vi "input.vi"(8 "error in":errorcluster, 10 "data table in":T1, 11 "Scan Engine runtime in":refnum<class "Scan Engine runtime.lvclass">) -> (0 "error out":errorcluster, 2 "data table out":T1, 3 "Scan Engine runtime out":refnum<class "Scan Engine runtime.lvclass">)   [LabVIEW 2015, in "Scan Engine runtime.lvclass"]
doc: "Provides an interface for reading data from a module at runtime. While this interface performs no operations, a child should provide an override which may read from any open sessions, references, or interfaces."
uses:
  Scan Engine runtime.lvclass
  <vilib>/NI/Tag Bus/table/data table.ctl
  Scan Engine runtime.lvclass/Scan Engine runtime.ctl
  <vilib>/NI/Tag Bus/table/data polymorphs/write one/write Double.vi
  <vilib>/NI/Tag Bus/table/data polymorphs/write one/write Single.vi
  <vilib>/NI/Tag Bus/table/data polymorphs/write one/write I64.vi
  <vilib>/NI/Tag Bus/table/data polymorphs/write one/write I32.vi
  <vilib>/NI/Tag Bus/table/data polymorphs/write one/write I16.vi
  <vilib>/NI/Tag Bus/table/data polymorphs/write one/write I8.vi
  <vilib>/NI/Tag Bus/table/data polymorphs/write one/write U64.vi
  <vilib>/NI/Tag Bus/table/data polymorphs/write one/write U32.vi
  <vilib>/NI/Tag Bus/table/data polymorphs/write one/write U16.vi
  <vilib>/NI/Tag Bus/table/data polymorphs/write one/write U8.vi
  <vilib>/NI/Tag Bus/table/data polymorphs/write one/write Boolean.vi
  <vilib>/NI/Tag Bus/table/data polymorphs/write many/write Doubles.vi
  <vilib>/NI/Tag Bus/table/data polymorphs/write many/write Singles.vi
  <vilib>/NI/Tag Bus/table/data polymorphs/write many/write I64s.vi
  <vilib>/NI/Tag Bus/table/data polymorphs/write many/write I32s.vi
  <vilib>/NI/Tag Bus/table/data polymorphs/write many/write I16s.vi
  <vilib>/NI/Tag Bus/table/data polymorphs/write many/write I8s.vi
  <vilib>/NI/Tag Bus/table/data polymorphs/write many/write U64s.vi
  <vilib>/NI/Tag Bus/table/data polymorphs/write many/write U32s.vi
  <vilib>/NI/Tag Bus/table/data polymorphs/write many/write U16s.vi
  <vilib>/NI/Tag Bus/table/data polymorphs/write many/write U8s.vi
  <vilib>/NI/Tag Bus/table/data polymorphs/write many/write Booleans.vi
  <vilib>/NI/Tag Bus/table/data table.lvlib
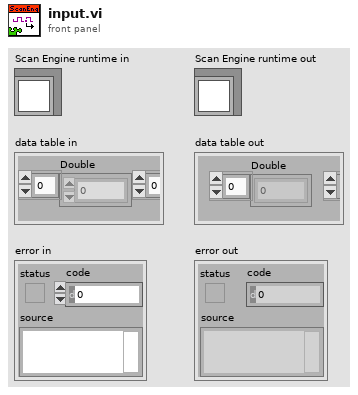
[diagram p1: front panel]
types:
  T1 = typedef "tag bus.lvlib/data table.lvlib/data table.ctl" = cluster{"Double":dbl[], "Single":sgl[], "I64":i64[], "I32":i32[], "I16":i16[], "I8":i8[], "U64":u64[], "U32":u32[], "U16":u16[], "U8":u8[], "Boolean":bool[], "String":string[], "Array of Double":cluster{"DBL Array":dbl[]}[], "Array of Single":cluster{"SGL Array":sgl[]}[], "Array of I64":cluster{"I64 Array":i64[]}[], "Array of I32":cluster{"I32 Array":i32[]}[], "Array of I16":cluster{"I16 Array":i16[]}[], "Array of I8":cluster{"I8 Array":i8[]}[], "Array of U64":cluster{"U64 Array":u64[]}[], "Array of U32":cluster{"U32 Array":u32[]}[], "Array of U16":cluster{"U16 Array":u16[]}[], "Array of U8":cluster{"U8 Array":u8[]}[], "Array of Boolean":cluster{"Boolean Array":bool[]}[], "Array of String":cluster{"String Array":string[]}[]}
  T2 = typedef "Scan Engine runtime.lvclass/IO_index_map.ctl" = cluster{"module_ref":refnum<k21>, "data type":T3, "IO_variable_info":T4[], "IO_module_index_array":i32[], "IO_table_index":i32[], "IO_table_index_ordered":i32[], "use_scanned_methods":bool}
  T3 = typedef "tag bus.lvlib/tag descriptor.lvclass/Data Type.ctl" = enum16{"Double", "Single", "I64", "I32", "I16", "I8", "U64", "U32", "U16", "U8", "Boolean", "String", "Array of Double", "Array of Single", "Array of I64", "Array of I32", "Array of I16", "Array of I8", "Array of U64", "Array of U32", "Array of U16", "Array of U8", "Array of Boolean", "Array of String"}
  T4 = typedef "Scan Engine runtime.lvclass/Index Map.ctl" = cluster{"data type":T3, "variable ref":refnum<k21>, "index":i32, "IO Var":bool, "module_index":i32}
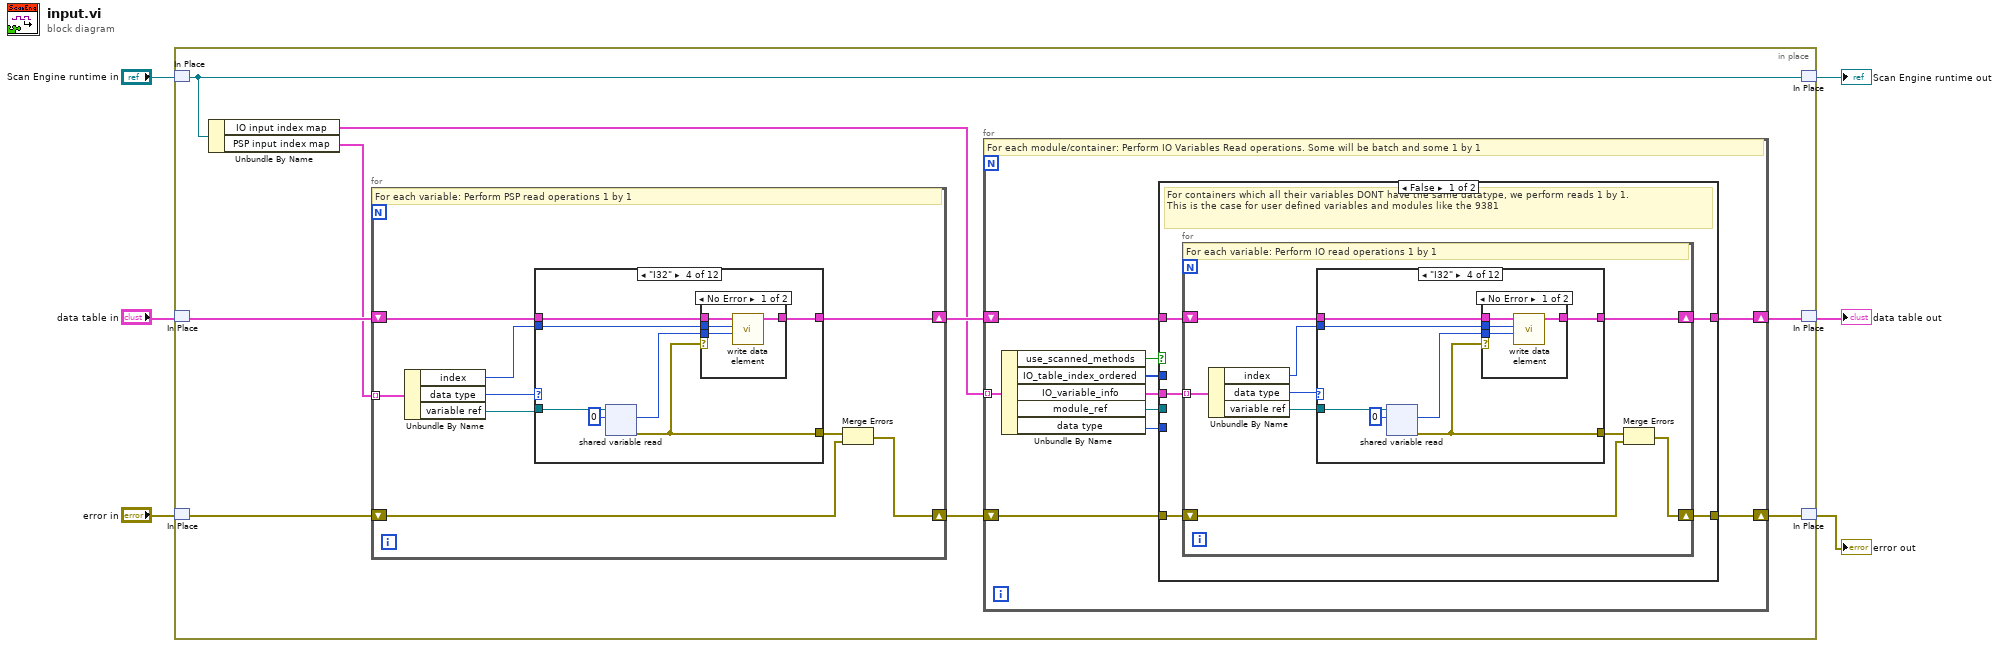
[diagram p0: block diagram]
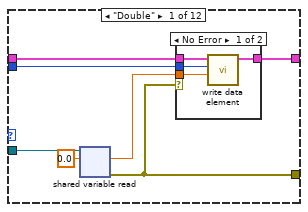
[diagram p2: hidden frame]
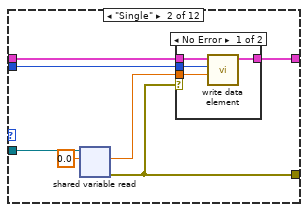
[diagram p4: hidden frame]
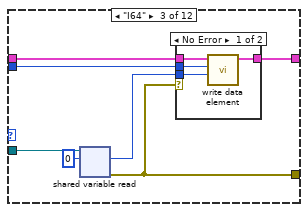
[diagram p6: hidden frame]
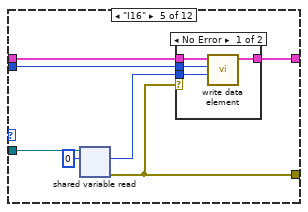
[diagram p9: hidden frame]
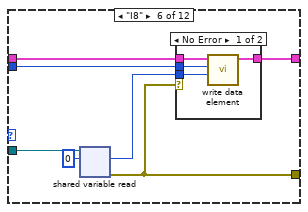
[diagram p11: hidden frame]
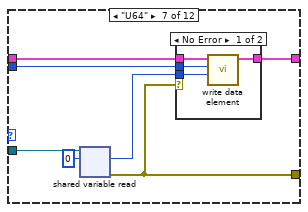
[diagram p13: hidden frame]
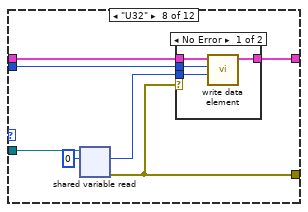
[diagram p15: hidden frame]
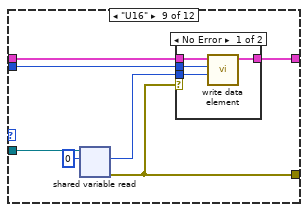
[diagram p17: hidden frame]
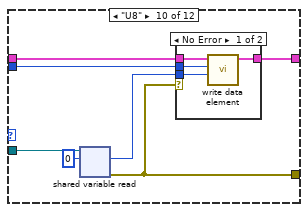
[diagram p19: hidden frame]
diagram:
  n1 = in-place {
    n2 = in-place-match #1("Scan Engine runtime in") -> (w15:refnum<class "Scan Engine runtime.lvclass">)
    n3 = in-place-match #2("data table in") -> (w14:T1)
    n4 = in-place-match #3("error in") -> (w13:errorcluster)
    n5 = Unbundle By Name(w15) -> ("IO input index map"=w10:T2[], "PSP input index map"=w9:T4[])
    n6 = for {
      shift-right: [w267] -> w12
      shift-left: w14 -> [w268]
      shift-right: [w262] -> w8
      shift-left: w13 -> [w263]
      tunnel: w9 -> [w270] mode=indexing
      # "For each variable: Perform PSP read operations 1 by 1"
      n7 = Unbundle By Name(w270) -> ("index"=w266:i32, "data type"=w269:T3, "variable ref"=w265:refnum<k21>)
      n8 = case shown="\"I32\"" w269 {
        tunnel: w268 -> [w277 w289 w301 w313 w325 w337 w349 w361 w373 w385 w397 w404]
        tunnel: [w276 w288 w300 w312 w324 w336 w348 w360 w372 w384 w396 w404] -> w267
        tunnel: w266 -> [w275 w287 w299 w311 w323 w335 w347 w359 w371 w383 w395 _]
        tunnel: w265 -> [w274 w286 w298 w310 w322 w334 w346 w358 w370 w382 w394 _]
        tunnel: [w271 w283 w295 w307 w319 w331 w343 w355 w367 w379 w391 errorcluster {"status"=FALSE, "code"=0, "source"=""} ("error IO")] -> w264
        frame "Double" {
          n9 = shared-variable-read(w274, 0.0) -> (w271:errorcluster, w272:dbl)  [unwired: 1 in, 1 out]
          n10 = case shown="No Error" w271 {
            tunnel: w277 -> [w281 w282]
            tunnel: [w280 w282] -> w276
            tunnel: w275 -> [w279 _]
            tunnel: w272 -> [w278 _]
            frame No Error {
              n11 = call-poly <vilib>:"write data element.vi"("value"=w278, "index"=w279, "data table in"=w281) -> ("data table out"=w280:T1)  [unwired: 8 in]
            }
            frame Error {
            }
          }
        }
        frame "Single" {
          n12 = shared-variable-read(w286, sgl 0.0) -> (w283:errorcluster, w284:sgl)  [unwired: 1 in, 1 out]
          n13 = case shown="No Error" w283 {
            tunnel: w289 -> [w293 w294]
            tunnel: [w292 w294] -> w288
            tunnel: w287 -> [w291 _]
            tunnel: w284 -> [w290 _]
            frame No Error {
              n14 = call-poly <vilib>:"write data element.vi"("value"=w290, "index"=w291, "data table in"=w293) -> ("data table out"=w292:T1)  [unwired: 8 in]
            }
            frame Error {
            }
          }
        }
        frame "I64" {
          n15 = shared-variable-read(w298, i64 0) -> (w295:errorcluster, w296:i64)  [unwired: 1 in, 1 out]
          n16 = case shown="No Error" w295 {
            tunnel: w301 -> [w305 w306]
            tunnel: [w304 w306] -> w300
            tunnel: w299 -> [w303 _]
            tunnel: w296 -> [w302 _]
            frame No Error {
              n17 = call-poly <vilib>:"write data element.vi"("value"=w302, "index"=w303, "data table in"=w305) -> ("data table out"=w304:T1)  [unwired: 8 in]
            }
            frame Error {
            }
          }
        }
        frame "I32" {
          n18 = shared-variable-read(w310, 0) -> (w307:errorcluster, w308:i32)  [unwired: 1 in, 1 out]
          n19 = case shown="No Error" w307 {
            tunnel: w313 -> [w317 w318]
            tunnel: [w316 w318] -> w312
            tunnel: w311 -> [w315 _]
            tunnel: w308 -> [w314 _]
            frame No Error {
              n20 = call-poly <vilib>:"write data element.vi"("value"=w314, "index"=w315, "data table in"=w317) -> ("data table out"=w316:T1)  [unwired: 8 in]
            }
            frame Error {
            }
          }
        }
        frame "I16" {
          n21 = shared-variable-read(w322, i16 0) -> (w319:errorcluster, w320:i16)  [unwired: 1 in, 1 out]
          n22 = case shown="No Error" w319 {
            tunnel: w325 -> [w329 w330]
            tunnel: [w328 w330] -> w324
            tunnel: w323 -> [w327 _]
            tunnel: w320 -> [w326 _]
            frame No Error {
              n23 = call-poly <vilib>:"write data element.vi"("value"=w326, "index"=w327, "data table in"=w329) -> ("data table out"=w328:T1)  [unwired: 8 in]
            }
            frame Error {
            }
          }
        }
        frame "I8" {
          n24 = shared-variable-read(w334, i8 0) -> (w331:errorcluster, w332:i8)  [unwired: 1 in, 1 out]
          n25 = case shown="No Error" w331 {
            tunnel: w337 -> [w341 w342]
            tunnel: [w340 w342] -> w336
            tunnel: w335 -> [w339 _]
            tunnel: w332 -> [w338 _]
            frame No Error {
              n26 = call-poly <vilib>:"write data element.vi"("value"=w338, "index"=w339, "data table in"=w341) -> ("data table out"=w340:T1)  [unwired: 8 in]
            }
            frame Error {
            }
          }
        }
        frame "U64" {
          n27 = shared-variable-read(w346, u64 0) -> (w343:errorcluster, w344:u64)  [unwired: 1 in, 1 out]
          n28 = case shown="No Error" w343 {
            tunnel: w349 -> [w353 w354]
            tunnel: [w352 w354] -> w348
            tunnel: w347 -> [w351 _]
            tunnel: w344 -> [w350 _]
            frame No Error {
              n29 = call-poly <vilib>:"write data element.vi"("value"=w350, "index"=w351, "data table in"=w353) -> ("data table out"=w352:T1)  [unwired: 8 in]
            }
            frame Error {
            }
          }
        }
        frame "U32" {
          n30 = shared-variable-read(w358, u32 0) -> (w355:errorcluster, w356:u32)  [unwired: 1 in, 1 out]
          n31 = case shown="No Error" w355 {
            tunnel: w361 -> [w365 w366]
            tunnel: [w364 w366] -> w360
            tunnel: w359 -> [w363 _]
            tunnel: w356 -> [w362 _]
            frame No Error {
              n32 = call-poly <vilib>:"write data element.vi"("value"=w362, "index"=w363, "data table in"=w365) -> ("data table out"=w364:T1)  [unwired: 8 in]
            }
            frame Error {
            }
          }
        }
        frame "U16" {
          n33 = shared-variable-read(w370, u16 0) -> (w367:errorcluster, w368:u16)  [unwired: 1 in, 1 out]
          n34 = case shown="No Error" w367 {
            tunnel: w373 -> [w377 w378]
            tunnel: [w376 w378] -> w372
            tunnel: w371 -> [w375 _]
            tunnel: w368 -> [w374 _]
            frame No Error {
              n35 = call-poly <vilib>:"write data element.vi"("value"=w374, "index"=w375, "data table in"=w377) -> ("data table out"=w376:T1)  [unwired: 8 in]
            }
            frame Error {
            }
          }
        }
        frame "U8" {
          n36 = shared-variable-read(w382, u8 0) -> (w379:errorcluster, w380:u8)  [unwired: 1 in, 1 out]
          n37 = case shown="No Error" w379 {
            tunnel: w385 -> [w389 w390]
            tunnel: [w388 w390] -> w384
            tunnel: w383 -> [w387 _]
            tunnel: w380 -> [w386 _]
            frame No Error {
              n38 = call-poly <vilib>:"write data element.vi"("value"=w386, "index"=w387, "data table in"=w389) -> ("data table out"=w388:T1)  [unwired: 8 in]
            }
            frame Error {
            }
          }
        }
        frame "Boolean" {
          n39 = shared-variable-read(w394, FALSE) -> (w391:errorcluster, w392:bool)  [unwired: 1 in, 1 out]
          n40 = case shown="No Error" w391 {
            tunnel: w397 -> [w401 w402]
            tunnel: [w400 w402] -> w396
            tunnel: w395 -> [w399 _]
            tunnel: w392 -> [w398 _]
            frame No Error {
              n41 = call-poly <vilib>:"write data element.vi"("value"=w398, "index"=w399, "data table in"=w401) -> ("data table out"=w400:T1)  [unwired: 8 in]
            }
            frame Error {
            }
          }
        }
        frame Default {
        }
      }
      n42 = Merge Errors(w264, w263) -> (w262:errorcluster)
    }
    n43 = for {
      shift-right: [w23] -> w11
      shift-left: w12 -> [w24]
      shift-right: [w21] -> w7
      shift-left: w8 -> [w22]
      tunnel: w10 -> [w25] mode=indexing
      # "For each module/container: Perform IO Variables Read operations. Some will be batch and some 1 by 1"
      n44 = Unbundle By Name(w25) -> ("use_scanned_methods"=w16:bool, "IO_table_index_ordered"=w18:i32[], "IO_variable_info"=w17:T4[], "module_ref"=w20:refnum<k21>, "data type"=w19:T3)
      n45 = case shown="False" w16 {
        tunnel: w24 -> [w26 w182]
        tunnel: [w27 w181] -> w23
        tunnel: w22 -> [w29 w179]
        tunnel: [w28 w178] -> w21
        tunnel: w20 -> [_ w177]
        tunnel: w19 -> [_ w176]
        tunnel: w18 -> [_ w175]
        tunnel: w17 -> [w30 w174]
        frame False {
          # "For containers which all their variables DONT have the same datatype, we perform reads 1 by 1.\nThis is the case for user defined variables and modules like the 9381"
          n46 = for {
            shift-right: [w36] -> w27
            shift-left: w26 -> [w37]
            shift-right: [w31] -> w28
            shift-left: w29 -> [w32]
            tunnel: w30 -> [w39] mode=indexing
            # "For each variable: Perform IO read operations 1 by 1"
            n47 = Unbundle By Name(w39) -> ("index"=w35:i32, "data type"=w38:T3, "variable ref"=w34:refnum<k21>)
            n48 = case shown="\"I32\"" w38 {
              tunnel: w37 -> [w46 w58 w70 w82 w94 w106 w118 w130 w142 w154 w166 w173]
              tunnel: [w45 w57 w69 w81 w93 w105 w117 w129 w141 w153 w165 w173] -> w36
              tunnel: w35 -> [w44 w56 w68 w80 w92 w104 w116 w128 w140 w152 w164 _]
              tunnel: w34 -> [w43 w55 w67 w79 w91 w103 w115 w127 w139 w151 w163 _]
              tunnel: [w40 w52 w64 w76 w88 w100 w112 w124 w136 w148 w160 errorcluster {"status"=FALSE, "code"=0, "source"=""} ("error IO")] -> w33
              frame "Double" {
                n49 = shared-variable-read(w43, 0.0) -> (w40:errorcluster, w41:dbl)  [unwired: 1 in, 1 out]
                n50 = case shown="No Error" w40 {
                  tunnel: w46 -> [w50 w51]
                  tunnel: [w49 w51] -> w45
                  tunnel: w44 -> [w48 _]
                  tunnel: w41 -> [w47 _]
                  frame No Error {
                    n51 = call-poly <vilib>:"write data element.vi"("value"=w47, "index"=w48, "data table in"=w50) -> ("data table out"=w49:T1)  [unwired: 8 in]
                  }
                  frame Error {
                  }
                }
              }
              frame "Single" {
                n52 = shared-variable-read(w55, sgl 0.0) -> (w52:errorcluster, w53:sgl)  [unwired: 1 in, 1 out]
                n53 = case shown="No Error" w52 {
                  tunnel: w58 -> [w62 w63]
                  tunnel: [w61 w63] -> w57
                  tunnel: w56 -> [w60 _]
                  tunnel: w53 -> [w59 _]
                  frame No Error {
                    n54 = call-poly <vilib>:"write data element.vi"("value"=w59, "index"=w60, "data table in"=w62) -> ("data table out"=w61:T1)  [unwired: 8 in]
                  }
                  frame Error {
                  }
                }
              }
              frame "I64" {
                n55 = shared-variable-read(w67, i64 0) -> (w64:errorcluster, w65:i64)  [unwired: 1 in, 1 out]
                n56 = case shown="No Error" w64 {
                  tunnel: w70 -> [w74 w75]
                  tunnel: [w73 w75] -> w69
                  tunnel: w68 -> [w72 _]
                  tunnel: w65 -> [w71 _]
                  frame No Error {
                    n57 = call-poly <vilib>:"write data element.vi"("value"=w71, "index"=w72, "data table in"=w74) -> ("data table out"=w73:T1)  [unwired: 8 in]
                  }
                  frame Error {
                  }
                }
              }
              frame "I32" {
                n58 = shared-variable-read(w79, 0) -> (w76:errorcluster, w77:i32)  [unwired: 1 in, 1 out]
                n59 = case shown="No Error" w76 {
                  tunnel: w82 -> [w86 w87]
                  tunnel: [w85 w87] -> w81
                  tunnel: w80 -> [w84 _]
                  tunnel: w77 -> [w83 _]
                  frame No Error {
                    n60 = call-poly <vilib>:"write data element.vi"("value"=w83, "index"=w84, "data table in"=w86) -> ("data table out"=w85:T1)  [unwired: 8 in]
                  }
                  frame Error {
                  }
                }
              }
              frame "I16" {
                n61 = shared-variable-read(w91, i16 0) -> (w88:errorcluster, w89:i16)  [unwired: 1 in, 1 out]
                n62 = case shown="No Error" w88 {
                  tunnel: w94 -> [w98 w99]
                  tunnel: [w97 w99] -> w93
                  tunnel: w92 -> [w96 _]
                  tunnel: w89 -> [w95 _]
                  frame No Error {
                    n63 = call-poly <vilib>:"write data element.vi"("value"=w95, "index"=w96, "data table in"=w98) -> ("data table out"=w97:T1)  [unwired: 8 in]
                  }
                  frame Error {
                  }
                }
              }
              frame "I8" {
                n64 = shared-variable-read(w103, i8 0) -> (w100:errorcluster, w101:i8)  [unwired: 1 in, 1 out]
                n65 = case shown="No Error" w100 {
                  tunnel: w106 -> [w110 w111]
                  tunnel: [w109 w111] -> w105
                  tunnel: w104 -> [w108 _]
                  tunnel: w101 -> [w107 _]
                  frame No Error {
                    n66 = call-poly <vilib>:"write data element.vi"("value"=w107, "index"=w108, "data table in"=w110) -> ("data table out"=w109:T1)  [unwired: 8 in]
                  }
                  frame Error {
                  }
                }
              }
              frame "U64" {
                n67 = shared-variable-read(w115, u64 0) -> (w112:errorcluster, w113:u64)  [unwired: 1 in, 1 out]
                n68 = case shown="No Error" w112 {
                  tunnel: w118 -> [w122 w123]
                  tunnel: [w121 w123] -> w117
                  tunnel: w116 -> [w120 _]
                  tunnel: w113 -> [w119 _]
                  frame No Error {
                    n69 = call-poly <vilib>:"write data element.vi"("value"=w119, "index"=w120, "data table in"=w122) -> ("data table out"=w121:T1)  [unwired: 8 in]
                  }
                  frame Error {
                  }
                }
              }
              frame "U32" {
                n70 = shared-variable-read(w127, u32 0) -> (w124:errorcluster, w125:u32)  [unwired: 1 in, 1 out]
                n71 = case shown="No Error" w124 {
                  tunnel: w130 -> [w134 w135]
                  tunnel: [w133 w135] -> w129
                  tunnel: w128 -> [w132 _]
                  tunnel: w125 -> [w131 _]
                  frame No Error {
                    n72 = call-poly <vilib>:"write data element.vi"("value"=w131, "index"=w132, "data table in"=w134) -> ("data table out"=w133:T1)  [unwired: 8 in]
                  }
                  frame Error {
                  }
                }
              }
              frame "U16" {
                n73 = shared-variable-read(w139, u16 0) -> (w136:errorcluster, w137:u16)  [unwired: 1 in, 1 out]
                n74 = case shown="No Error" w136 {
                  tunnel: w142 -> [w146 w147]
                  tunnel: [w145 w147] -> w141
                  tunnel: w140 -> [w144 _]
                  tunnel: w137 -> [w143 _]
                  frame No Error {
                    n75 = call-poly <vilib>:"write data element.vi"("value"=w143, "index"=w144, "data table in"=w146) -> ("data table out"=w145:T1)  [unwired: 8 in]
                  }
                  frame Error {
                  }
                }
              }
              frame "U8" {
                n76 = shared-variable-read(w151, u8 0) -> (w148:errorcluster, w149:u8)  [unwired: 1 in, 1 out]
                n77 = case shown="No Error" w148 {
                  tunnel: w154 -> [w158 w159]
                  tunnel: [w157 w159] -> w153
                  tunnel: w152 -> [w156 _]
                  tunnel: w149 -> [w155 _]
                  frame No Error {
                    n78 = call-poly <vilib>:"write data element.vi"("value"=w155, "index"=w156, "data table in"=w158) -> ("data table out"=w157:T1)  [unwired: 8 in]
                  }
                  frame Error {
                  }
                }
              }
              frame "Boolean" {
                n79 = shared-variable-read(w163, FALSE) -> (w160:errorcluster, w161:bool)  [unwired: 1 in, 1 out]
                n80 = case shown="No Error" w160 {
                  tunnel: w166 -> [w170 w171]
                  tunnel: [w169 w171] -> w165
                  tunnel: w164 -> [w168 _]
                  tunnel: w161 -> [w167 _]
                  frame No Error {
                    n81 = call-poly <vilib>:"write data element.vi"("value"=w167, "index"=w168, "data table in"=w170) -> ("data table out"=w169:T1)  [unwired: 8 in]
                  }
                  frame Error {
                  }
                }
              }
              frame Default {
              }
            }
            n82 = Merge Errors(w33, w32) -> (w31:errorcluster)
          }
        }
        frame True {
          # "For containers which all their variables have the same datatype, we perform a batch read"
          n83 = case shown="\"Single\"" w176 {
            tunnel: w182 -> [w185 w192 w199 w206 w213 w220 w227 w234 w241 w248 w255 w261]
            tunnel: [w186 w193 w200 w207 w214 w221 w228 w235 w242 w249 w256 w261] -> w181
            tunnel: w177 -> [w189 w196 w203 w210 w217 w224 w231 w238 w245 w252 w259 _]
            tunnel: [w188 w195 w202 w209 w216 w223 w230 w237 w244 w251 w258 errorcluster {"status"=FALSE, "code"=0, "source"=""} ("error IO")] -> w180
            tunnel: w175 -> [w184 w191 w198 w205 w212 w219 w226 w233 w240 w247 w254 _]
            tunnel: w174 -> [_ _ _ _ _ _ _ _ _ _ _ _]
            frame "Double" {
              n84 = shared-variable-read(w189, dbl[] []) -> (w188:errorcluster, w183:dbl[])  [unwired: 1 in, 1 out]
              n85 = call-poly <vilib>:"write multiple elements.vi"("values"=w183, "indices"=w184, "data table in"=w185) -> ("data table out"=w186:T1)  [unwired: 8 in]
            }
            frame "Single" {
              n86 = shared-variable-read(w196, sgl[] []) -> (w195:errorcluster, w190:sgl[])  [unwired: 1 in, 1 out]
              n87 = call-poly <vilib>:"write multiple elements.vi"("values"=w190, "indices"=w191, "data table in"=w192) -> ("data table out"=w193:T1)  [unwired: 8 in]
            }
            frame "I64" {
              n88 = shared-variable-read(w203, i64[] []) -> (w202:errorcluster, w197:i64[])  [unwired: 1 in, 1 out]
              n89 = call-poly <vilib>:"write multiple elements.vi"("values"=w197, "indices"=w198, "data table in"=w199) -> ("data table out"=w200:T1)  [unwired: 8 in]
            }
            frame "I32" {
              n90 = shared-variable-read(w210, i32[] []) -> (w209:errorcluster, w204:i32[])  [unwired: 1 in, 1 out]
              n91 = call-poly <vilib>:"write multiple elements.vi"("values"=w204, "indices"=w205, "data table in"=w206) -> ("data table out"=w207:T1)  [unwired: 8 in]
            }
            frame "I16" {
              n92 = shared-variable-read(w217, i16[] []) -> (w216:errorcluster, w211:i16[])  [unwired: 1 in, 1 out]
              n93 = call-poly <vilib>:"write multiple elements.vi"("values"=w211, "indices"=w212, "data table in"=w213) -> ("data table out"=w214:T1)  [unwired: 8 in]
            }
            frame "I8" {
              n94 = shared-variable-read(w224, i8[] []) -> (w223:errorcluster, w218:i8[])  [unwired: 1 in, 1 out]
              n95 = call-poly <vilib>:"write multiple elements.vi"("values"=w218, "indices"=w219, "data table in"=w220) -> ("data table out"=w221:T1)  [unwired: 8 in]
            }
            frame "U64" {
              n96 = shared-variable-read(w231, u64[] []) -> (w230:errorcluster, w225:u64[])  [unwired: 1 in, 1 out]
              n97 = call-poly <vilib>:"write multiple elements.vi"("values"=w225, "indices"=w226, "data table in"=w227) -> ("data table out"=w228:T1)  [unwired: 8 in]
            }
            frame "U32" {
              n98 = shared-variable-read(w238, u32[] []) -> (w237:errorcluster, w232:u32[])  [unwired: 1 in, 1 out]
              n99 = call-poly <vilib>:"write multiple elements.vi"("values"=w232, "indices"=w233, "data table in"=w234) -> ("data table out"=w235:T1)  [unwired: 8 in]
            }
            frame "U16" {
              n100 = shared-variable-read(w245, u16[] []) -> (w244:errorcluster, w239:u16[])  [unwired: 1 in, 1 out]
              n101 = call-poly <vilib>:"write multiple elements.vi"("values"=w239, "indices"=w240, "data table in"=w241) -> ("data table out"=w242:T1)  [unwired: 8 in]
            }
            frame "U8" {
              n102 = shared-variable-read(w252, u8[] []) -> (w251:errorcluster, w246:u8[])  [unwired: 1 in, 1 out]
              n103 = call-poly <vilib>:"write multiple elements.vi"("values"=w246, "indices"=w247, "data table in"=w248) -> ("data table out"=w249:T1)  [unwired: 8 in]
            }
            frame "Boolean" {
              n104 = shared-variable-read(w259, bool[] []) -> (w258:errorcluster, w253:bool[])  [unwired: 1 in, 1 out]
              n105 = call-poly <vilib>:"write multiple elements.vi"("values"=w253, "indices"=w254, "data table in"=w255) -> ("data table out"=w256:T1)  [unwired: 8 in]
            }
            frame Default {
            }
          }
          n106 = Merge Errors(w180, w179) -> (w178:errorcluster)
        }
      }
    }
    n107 = in-place-match #1(w15) -> (→"Scan Engine runtime out":refnum<class "Scan Engine runtime.lvclass">)
    n108 = in-place-match #2(w11) -> (→"data table out":T1)
    n109 = in-place-match #3(w7) -> (→"error out":errorcluster)
  }
